vi "configuration UI.vi"() -> ()   [LabVIEW 2015, in "Scan Engine editor node.lvclass"]
uses:
  Scan Engine editor node.lvclass
  <vilib>/NI/Configuration Framework/Node/NodeRef.ctl
  <vilib>/NI/Configuration Framework/Node/NISE_CEF_Node.lvclass
  <vilib>/NI/AMC/Message Queue.ctl
  <vilib>/NI/AMC/Message.ctl
  <vilib>/NI/Tools/Keyed Array/KeyedArray.ctl
  <vilib>/NI/Configuration Framework/Node/UserEventRef.ctl
  <vilib>/NI/Configuration Framework/Controls/EventCluster.ctl
  <vilib>/NI/DCAF UI Toolkit/Controls/Configure.ctl
  <vilib>/NI/DCAF UI Toolkit/Controls/Add.ctl
  <vilib>/NI/DCAF UI Toolkit/Controls/Remove.ctl
  <vilib>/NI/Configuration Framework/Node/StopEvent.ctl
  <vilib>/NI/Configuration Framework/Node/RefreshUIEvent.ctl
  <vilib>/NI/Configuration Framework/Node/CacheState.ctl
  <vilib>/NI/Configuration Framework/Node/NodeChangeEvent.ctl
  <vilib>/NI/Tag Bus/tag/Data Type.ctl
  Permissions Enum.ctl
  <vilib>/NI/DCAF/Tag Editor Core/Table API/Available Tag Menu/channel action event.ctl
  <vilib>/NI/DCAF/Tag Editor Core/Table API/Available Tag Menu/dialog output action.ctl
  <vilib>/NI/Tag Bus Module Framework/channel/TBM channel.lvclass
  <vilib>/NI/Tag Bus/tag/tag descriptor.lvclass
  <vilib>/NI/DCAF/Tag Editor Core/Table API/Table Manager/Call Back Ref Type Def.ctl
  <vilib>/NI/DCAF/Tag Editor Core/Configuration Editor/Classes/Engine Parent/Engine Parent Editor Node.lvclass
  <vilib>/NI/DCAF/Tag Editor Core/Configuration Editor/Classes/Module editor node/module editor node.lvclass
  <vilib>/NI/DCAF UI Toolkit/Controls/Import.ctl
  <vilib>/NI/DCAF UI Toolkit/Controls/Export.ctl
  <vilib>/NI/DCAF/Tag Editor Core/Table API/Table Manager/references.ctl
  <vilib>/Utility/miscctls.llb/LVPositionTypeDef.ctl
  <vilib>/NI/DCAF/Tag Editor Core/Table API/Listbox/Multi Column Listbox.lvclass
  configuration/Scan Engine configuration.lvclass
  <vilib>/NI/Configuration Framework/NISE_CEF_TreeControl.lvlib
  <vilib>/NI/Tools/Keyed Array/Tools_KeyedArray.lvlib
  <vilib>/NI/AMC/AMC.lvlib
  <vilib>/NI/DCAF/Tag Editor Core/Table API/Table Manager.lvlib
  <vilib>/NI/DCAF/Tag Editor Core/Table API/Table Manager/Table Manager.lvclass
  <vilib>/NI/DCAF UI Toolkit/Controls/DCAF UI Elements.lvlib
panel:
  in  "user event out":refnum<user-event>
  in  "Permissions":T1
  in  "data type":T2
  in  "node change":T3
  in  "cache state":T4
  in  "refresh UI":T5
  in  "stop event":T6
  in  "Tab Control":enum32{"Scan Engine Settings", "Import Export"}(tab)
  in  "Overwrite scan engine config":bool
  in  "Remove Button":T7
  in  "Add Button":T8
  in  "Table":i32(listbox)=13
  in  "settings":T9
  in  "Scan Period (uSec)":u32
  in  "Discover Channels?":bool
  in  "Import":T10
  in  "Generate Tags":bool
  in  "Import from csv":T10
  in  "Export":T11
  in  "user event":T12
  in  "main queue":T13
  in  "node ref":T14
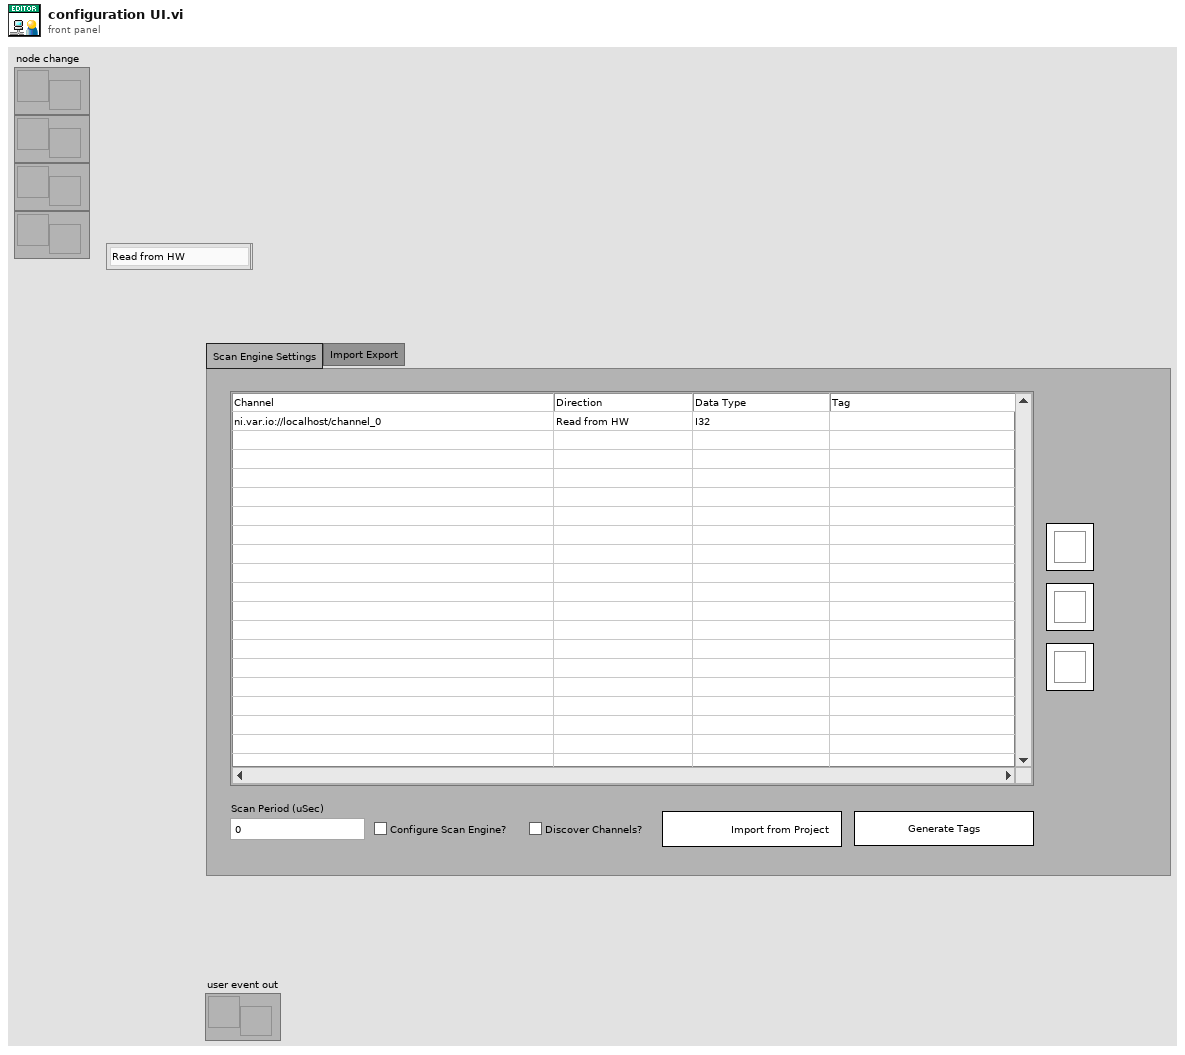
[diagram p1: front panel]
types:
  T1 = typedef "Scan Engine editor node.lvclass/Permissions Enum.ctl" = enum16{"Read from HW", "Write to HW"}
  T2 = typedef "tag bus.lvlib/tag descriptor.lvclass/Data Type.ctl" = enum16{"Double", "Single", "I64", "I32", "I16", "I8", "U64", "U32", "U16", "U8", "Boolean", "String", "Array of Double", "Array of Single", "Array of I64", "Array of I32", "Array of I16", "Array of I8", "Array of U64", "Array of U32", "Array of U16", "Array of U8", "Array of Boolean", "Array of String"}
  T3 = typedef "NISE_CEF_Node.lvclass/NodeChangeEvent.ctl" = refnum<user-event>
  T4 = typedef "NISE_CEF_Node.lvclass/CacheState.ctl" = refnum<user-event>
  T5 = typedef "NISE_CEF_Node.lvclass/RefreshUIEvent.ctl" = refnum<user-event>
  T6 = typedef "NISE_CEF_Node.lvclass/StopEvent.ctl" = refnum<user-event>
  T7 = typedef "DCAF UI Elements.lvlib/Remove.ctl" = bool
  T8 = typedef "DCAF UI Elements.lvlib/Add.ctl" = bool
  T9 = typedef "DCAF UI Elements.lvlib/Configure.ctl" = bool
  T10 = typedef "DCAF UI Elements.lvlib/Import.ctl" = bool
  T11 = typedef "DCAF UI Elements.lvlib/Export.ctl" = bool
  T12 = typedef "NISE_CEF_Node.lvclass/UserEventRef.ctl" = refnum<user-event>
  T13 = typedef "AMC.lvlib/Message Queue.ctl" = refnum<queue>
  T14 = typedef "NISE_CEF_Node.lvclass/NodeRef.ctl" = refnum<data-value>
  T15 = typedef "Table Manager.lvlib/Table Manager.lvclass/references.ctl" = cluster{"stop event":T6, "refresh UI":T5, "cache state":T4, "node change":T3, "user event out":refnum<user-event>, "main queue":T13, "user event":T12}
  T16 = typedef "LVPositionTypeDef.ctl" = cluster{"Left":i32, "Top":i32}
  T17 = typedef "Table Manager.lvlib/Table Manager.lvclass/object ref.ctl" = cluster{"engine":refnum<data-value>, "Node Ref":refnum<data-value>}
  T18 = typedef "Table Manager.lvlib/Column.lvclass/Column Descriptor.ctl" = cluster{"name":string, "caption":string, "Column Type":T19, "Params":string, "AutoSizeMode":i32, "FillWeight":sgl, "MinWidth":u32, "tooltip":string, "Enum Reference":refnum<vi>, "Channel suffix":string, "Read Only":bool, "Call Back VI":T20, "DT Dependency":i32, "name dependency":i32, "data type":T2, "Custom Column":refnum<class "Column.lvclass">}
  T19 = typedef "Table Manager.lvlib/Column.lvclass/Column Type.ctl" = enum16{"String", "Mapping", "Enum", "Custom"}
  T20 = typedef "Table Manager.lvlib/Table Manager.lvclass/Call Back Ref Type Def.ctl" = refnum<vi>
  T21 = typedef "Table Manager.lvlib/Table Manager.lvclass/Table Events.ctl" = cluster{"Menu Selection":refnum<user-event>}
  T22 = enum8{"Enabled", "Disabled", "Disabled and Grayed Out"}
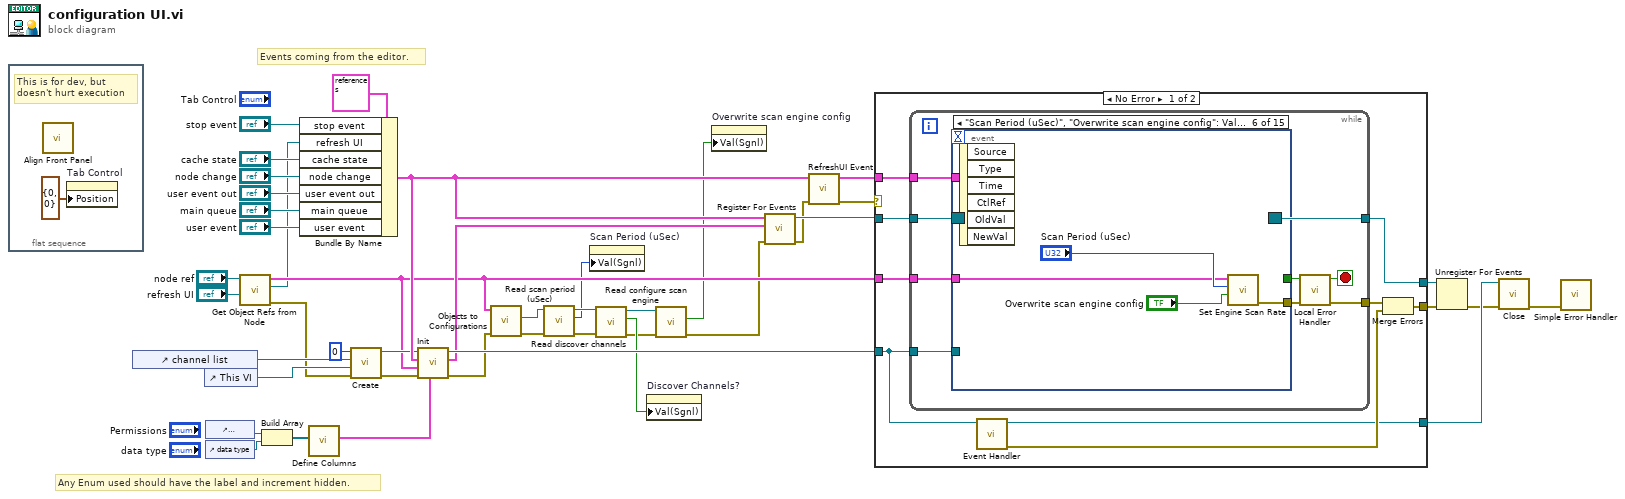
[diagram p0: block diagram]
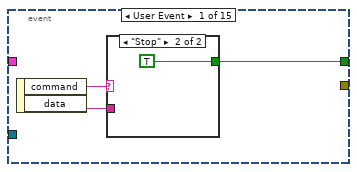
[diagram p2: hidden frame]
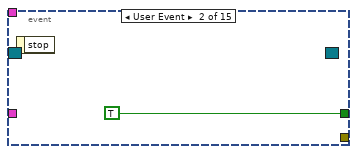
[diagram p4: hidden frame]
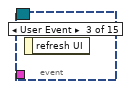
[diagram p5: hidden frame]
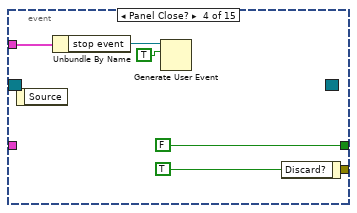
[diagram p6: hidden frame]
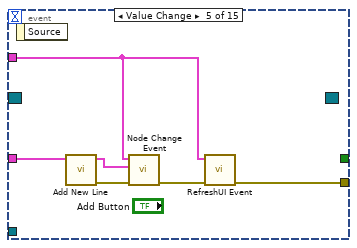
[diagram p7: hidden frame]
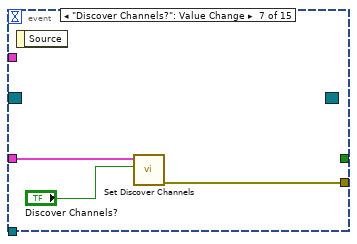
[diagram p8: hidden frame]
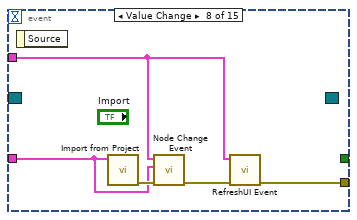
[diagram p9: hidden frame]
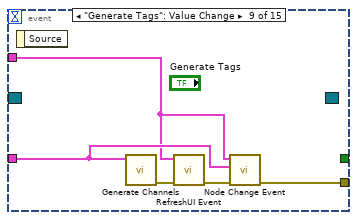
[diagram p10: hidden frame]
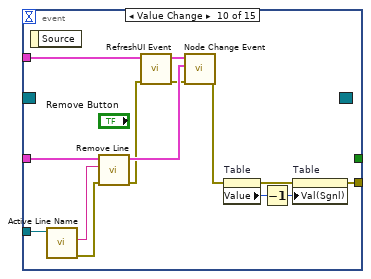
[diagram p11: hidden frame]
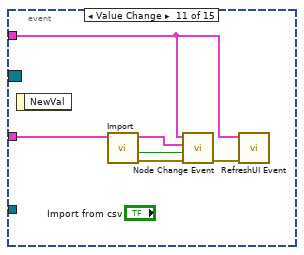
[diagram p12: hidden frame]
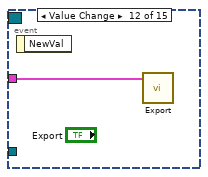
[diagram p13: hidden frame]
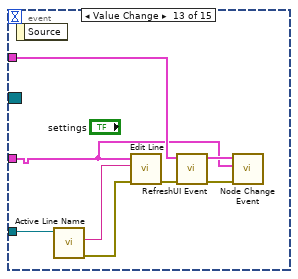
[diagram p14: hidden frame]
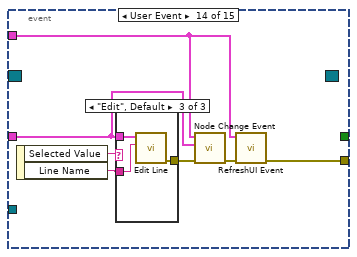
[diagram p15: hidden frame]
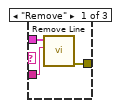
[diagram p16: hidden frame]
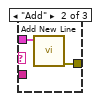
[diagram p17: hidden frame]
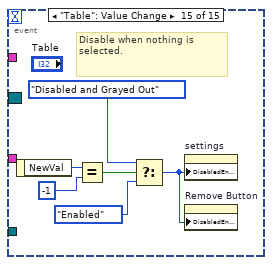
[diagram p18: hidden frame]
diagram:
  # "Any Enum used should have the label and increment hidden."
  # "Events coming from the editor."
  n1 = flat-sequence {
    frame #0 {
      # "This is for dev, but doesn't hurt execution"
      n2 = call <vilib>:"Align Front Panel.vi"() -> ()  [unwired: 10 in, 2 out]
      n3 = property on="Tab Control" class="TabCtl (strict)"("Position"=T16 {"Left"=0, "Top"=0}) -> ()  [unwired: 2 in, 2 out]
    }
  }
  n4 = control-ref of="channel list"() -> (w24:refnum<vi>)
  n5 = control-ref of="This VI"() -> (w22:refnum<vi>)
  n6 = control-ref of="Permissions"() -> (w31:refnum<vi>)
  n7 = control-ref of="data type"() -> (w30:refnum<vi>)
  n8 = call "Get Object Refs from Node.vi"("refresh UI"="refresh UI", "Data Value Reference in"="node ref") -> ("error out"=w6:errorcluster, "refresh UI out"=w7:T5, "references"=w18:T17)  [unwired: 7 in]
  n9 = Build Array(w31, w30) -> (w29:refnum<vi>[])
  n10 = Bundle By Name(cluster=T15 {"stop event"=refnum, "refresh UI"=refnum, "cache state"=refnum, "node change"=refnum, "user event out"=refnum, "main queue"=refnum, "user event"=refnum} ("References"), "stop event"="stop event", "refresh UI"=w7, "cache state"="cache state", "node change"="node change", "user event out"="user event out", "main queue"="main queue", "user event"="user event") -> (w32:T15)
  n11 = call "Define Columns.vi"("Enum Array"=w29) -> ("Column Definition"=w34:T18[])  [unwired: 10 in]
  n12 = call <vilib>:"Create.vi"("error in (no error)"=w6, "Top VI"=w22, "Listbox"=w24, "Index"=0) -> ("error out"=w5:errorcluster, "reference out"=w21:refnum<class "Multi Column Listbox.lvclass">)  [unwired: 6 in]
  n13 = call-dynamic "Init.vi"("Column Descriptors"=w34, "error in (no error)"=w5, "Node object refs"=w18, "Event References"=w32, "Multi Column Listbox in"=w21) -> ("error out"=w20:errorcluster, "Table Events"=w19:T21, "Multi Column Listbox out"=w28:refnum<class "Multi Column Listbox.lvclass">)  [unwired: 4 in]
  n14 = call "Objects to Configurations.vi"("error in (no error)"=w20, "Objects in"=w18) -> ("error out"=w14:errorcluster, "tag bus configurable plugin module configuration"=w17:refnum<class "Scan Engine configuration.lvclass">)  [unwired: 7 in, 1 out]
  n15 = call-dynamic "Read scan period (uSec).vi"("error in (no error)"=w14, "Scan Engine configuration1 in"=w17) -> ("error out"=w15:errorcluster, "scan period (uSec)"=w13:u32, "Scan Engine configuration1 out"=w16:refnum<class "Scan Engine configuration.lvclass">)  [unwired: 7 in]
  n16 = property on="Scan Period (uSec)" class="DigNum (strict)"("Val(Sgnl)"=w13) -> ()  [unwired: 2 in, 2 out]
  n17 = call-dynamic "Read discover channels.vi"("error in (no error)"=w15, "Scan Engine configuration1 in"=w16) -> ("error out"=w4:errorcluster, "discover channels"=w12:bool, "Scan Engine configuration1 out"=w3:refnum<class "Scan Engine configuration.lvclass">)  [unwired: 7 in]
  n18 = property on="Discover Channels?" class="Bool (strict)"("Val(Sgnl)"=w12) -> ()  [unwired: 2 in, 2 out]
  n19 = call-dynamic "Read configure scan engine.vi"("error in (no error)"=w4, "Scan Engine configuration1 in"=w3) -> ("error out"=w2:errorcluster, "configure scan engine"=w1:bool)  [unwired: 7 in, 1 out]
  n20 = property on="Overwrite scan engine config" class="Bool (strict)"("Val(Sgnl)"=w1) -> ()  [unwired: 2 in, 2 out]
  n21 = call "Register For Events.vi"("error in"=w2, "Table Events"=w19, "References"=w32) -> ("error out"=w26:errorcluster, "Event Registration Refnum"=w35:refnum<event-registration>)  [unwired: 7 in]
  n22 = call "RefreshUI Event.vi"("error in (no error)"=w26, "References in"=w32) -> ("error out"=w25:errorcluster, "References out"=w33:T15)  [unwired: 8 in]
  n23 = case shown="No Error" w25 {
    selector: w25 -> [_ w147]
    tunnel: w35 -> [w54 w146]
    tunnel: [w53 w146] -> w44
    tunnel: [w47 w147] -> w43
    tunnel: w33 -> [w52 _]
    tunnel: w18 -> [w51 _]
    tunnel: w28 -> [w50 w145]
    tunnel: [w46 w145] -> w11
    frame No Error {
      n24 = while {
        tunnel: w54 -> [w63]
        tunnel: [w62] -> w53
        tunnel: [w59] -> w48
        tunnel: w52 -> [w57]
        tunnel: w51 -> [w56]
        tunnel: w50 -> [w55]
        stop <- w61 stop-if-true
        n25 = event shown="[5] \"Scan Period (uSec)\", \"Overwrite scan engine config\": Value Change" {
          selector: w63 -> [_ _ _ _ _ _ _ _ _ _ _ _ _ _ _]
          dyn-events: [_ _ _ _ _ _ _ _ _ _ _ _ _ _ _] -> w62
          timeout: _ -> [_ _ _ _ _ _ _ _ _ _ _ _ _ _ _]
          tunnel: [w66 TRUE _ FALSE _ _ _ _ _ _ _ _ _ _ _] -> w60
          tunnel: [_ _ _ _ w74 w80 w83 w88 w91 w96 _ _ _ w128 _] -> w58
          tunnel: w57 -> [_ _ _ w70 w77 _ _ w87 w92 w108 w110 _ w118 w124 _]
          tunnel: w56 -> [_ _ _ _ w78 w81 w85 w86 w93 w107 w114 w115 w117 w125 _]
          tunnel: w55 -> [_ _ _ _ _ _ _ _ _ w103 _ _ w123 _ _]
          event User Event {
            n26 = event-data() -> ("command"=w65:string, "data"=w64:string)  [unwired: 1 in]
            n27 = case shown="\"Stop\"" w65 {
              tunnel: [_ TRUE] -> w66
              tunnel: w64 -> [_ _]
              frame Default {
              }
              frame "Stop" {
              }
            }
          }
          event User Event {
            n28 = event-data() -> ()  [unwired: 1 in, 1 out]
          }
          event User Event {
            n29 = event-data() -> ()  [unwired: 1 in, 1 out]
          }
          event Panel Close? {
            n30 = event-data() -> ()  [unwired: 1 in, 1 out]
            n31 = Unbundle By Name(w70) -> ("stop event"=w69:T6)
            n32 = Generate User Event(user event=w69, event data cluster=TRUE ("event data")) -> ()  [unwired: 2 in, 2 out]
            n33 = event-data("Discard?"=TRUE) -> ()  [unwired: 1 in, 1 out]
          }
          event Value Change {
            n34 = event-data() -> ()  [unwired: 1 in, 1 out]
            n35 = call "Add New Line.vi"("objects"=w78) -> ("error out"=w76:errorcluster)  [unwired: 9 in, 1 out]
            n36 = call "Node Change Event.vi"("error in (no error)"=w76, "objects"=w78, "References in"=w77) -> ("error out"=w75:errorcluster)  [unwired: 8 in]
            n37 = call "RefreshUI Event.vi"("error in (no error)"=w75, "References in"=w77) -> ("error out"=w74:errorcluster)  [unwired: 8 in, 1 out]
          }
          event "Scan Period (uSec)", "Overwrite scan engine config": Value Change {
            n38 = event-data() -> ()  [unwired: 1 in, 6 out]
            n39 = call "Set Engine Scan Rate.vi"("Configure Scan Engine"="Overwrite scan engine config", "scan period (uSec)"="Scan Period (uSec)", "references in"=w81) -> ("error out"=w80:errorcluster)  [unwired: 7 in, 1 out]
          }
          event "Discover Channels?": Value Change {
            n40 = event-data() -> ()  [unwired: 1 in, 1 out]
            n41 = call "Set Discover Channels.vi"("discover channels"="Discover Channels?", "references in"=w85) -> ("error out"=w83:errorcluster)  [unwired: 8 in, 1 out]
          }
          event Value Change {
            n42 = event-data() -> ()  [unwired: 1 in, 1 out]
            n43 = call "Import from Project.vi"("references"=w86) -> ("error out"=w90:errorcluster)  [unwired: 9 in, 1 out]
            n44 = call "Node Change Event.vi"("error in (no error)"=w90, "objects"=w86, "References in"=w87) -> ("error out"=w89:errorcluster)  [unwired: 8 in]
            n45 = call "RefreshUI Event.vi"("error in (no error)"=w89, "References in"=w87) -> ("error out"=w88:errorcluster)  [unwired: 8 in, 1 out]
          }
          event "Generate Tags": Value Change {
            n46 = event-data() -> ()  [unwired: 1 in, 1 out]
            n47 = call "Generate Channels.vi"("references in"=w93) -> ("error out"=w94:errorcluster)  [unwired: 10 in]
            n48 = call "RefreshUI Event.vi"("error in (no error)"=w94, "References in"=w92) -> ("error out"=w95:errorcluster)  [unwired: 8 in, 1 out]
            n49 = call "Node Change Event.vi"("error in (no error)"=w95, "objects"=w93, "References in"=w92) -> ("error out"=w91:errorcluster)  [unwired: 8 in]
          }
          event Value Change {
            n50 = event-data() -> ()  [unwired: 1 in, 1 out]
            n51 = call-dynamic "Active Line Name.vi"("Multi Column Listbox in"=w103) -> ("error out"=w101:errorcluster, "Active Line Name"=w102:string)  [unwired: 8 in, 1 out]
            n52 = call "Remove Line.vi"("error in"=w101, "Active Line Name"=w102, "Objects"=w107) -> ("error out"=w104:errorcluster)  [unwired: 8 in]
            n53 = call "RefreshUI Event.vi"("error in (no error)"=w104, "References in"=w108) -> ("error out"=w106:errorcluster, "References out"=w105:T15)  [unwired: 8 in]
            n54 = call "Node Change Event.vi"("error in (no error)"=w106, "objects"=w107, "References in"=w105) -> ("error out"=w98:errorcluster)  [unwired: 8 in]
            n55 = property on="Table" class="MCListbox (strict)"(error in=w98) -> (error out=w97:errorcluster, "Value"=w100:i32)  [unwired: 1 in, 1 out]
            n56 = Decrement(x=w100) -> (x-1=w99:i32)
            n57 = property on="Table" class="MCListbox (strict)"(error in=w97, "Val(Sgnl)"=w99) -> (error out=w96:errorcluster)  [unwired: 1 in, 1 out]
          }
          event Value Change {
            n58 = event-data() -> ()  [unwired: 1 in, 1 out]
            n59 = call "Import.vi"("Objects in"=w114) -> ("error out"=w113:errorcluster, "Update"=w112:bool, "Objects out"=w111:T17)  [unwired: 8 in]
            n60 = call "Node Change Event.vi"("error in (no error)"=w113, "Send (T)"=w112, "objects"=w111, "References in"=w110) -> ("error out"=w109:errorcluster)  [unwired: 7 in]
            n61 = call "RefreshUI Event.vi"("error in (no error)"=w109, "References in"=w110) -> ()  [unwired: 8 in, 2 out]
          }
          event Value Change {
            n62 = event-data() -> ()  [unwired: 1 in, 1 out]
            n63 = call "Export.vi"("Objects"=w115) -> ()  [unwired: 10 in, 1 out]
          }
          event Value Change {
            n64 = event-data() -> ()  [unwired: 1 in, 1 out]
            n65 = call-dynamic "Active Line Name.vi"("Multi Column Listbox in"=w123) -> ("error out"=w121:errorcluster, "Active Line Name"=w122:string)  [unwired: 8 in, 1 out]
            n66 = call "Edit Line.vi"("error in"=w121, "Line Name"=w122, "References"=w117) -> ("error out"=w116:errorcluster)  [unwired: 7 in, 1 out]
            n67 = call "RefreshUI Event.vi"("error in (no error)"=w116, "References in"=w118) -> ("error out"=w119:errorcluster, "References out"=w120:T15)  [unwired: 8 in]
            n68 = call "Node Change Event.vi"("error in (no error)"=w119, "objects"=w117, "References in"=w120) -> ()  [unwired: 8 in, 1 out]
          }
          event User Event {
            n69 = event-data() -> ("Selected Value"=w130:string, "Line Name"=w127:string)  [unwired: 1 in]
            n70 = case shown="\"Edit\", Default" w130 {
              tunnel: w127 -> [w133 _ w138]
              tunnel: w125 -> [w132 w135 w137]
              tunnel: [w131 w134 w136] -> w126
              frame "Remove" {
                n71 = call "Remove Line.vi"("Active Line Name"=w133, "Objects"=w132) -> ("error out"=w131:errorcluster)  [unwired: 9 in]
              }
              frame "Add" {
                n72 = call "Add New Line.vi"("objects"=w135) -> ("error out"=w134:errorcluster)  [unwired: 9 in, 1 out]
              }
              frame "Edit", Default {
                n73 = call "Edit Line.vi"("Line Name"=w138, "References"=w137) -> ("error out"=w136:errorcluster)  [unwired: 8 in, 1 out]
              }
            }
            n74 = call "Node Change Event.vi"("error in (no error)"=w126, "objects"=w125, "References in"=w124) -> ("error out"=w129:errorcluster)  [unwired: 8 in]
            n75 = call "RefreshUI Event.vi"("error in (no error)"=w129, "References in"=w124) -> ("error out"=w128:errorcluster)  [unwired: 8 in, 1 out]
          }
          event "Table": Value Change {
            # "Disable when nothing is selected."
            n76 = event-data() -> ("NewVal"=w144:i32)  [unwired: 1 in]
            n77 = Equal?(x=w144, y=-1) -> (x = y?=w142:bool)
            n78 = Select(t=T22."Disabled and Grayed Out" ("Disabled"), s=w142, f=T22."Enabled" ("Disabled")) -> (s? t:f=w140:T22)
            n79 = property on="settings" class="Bool"("DisabledEnum"=w140) -> ()  [unwired: 2 in, 2 out]
            n80 = property on="Remove Button" class="Bool"("DisabledEnum"=w140) -> ()  [unwired: 2 in, 2 out]
          }
        }
        n81 = call "Local Error Handler.vi"("error in"=w58, "Stop in"=w60) -> ("error out"=w59:errorcluster, "Stop out"=w61:bool)  [unwired: 8 in]
      }
      n82 = call-dynamic "Event Handler.vi"("Listbox in"=w50) -> ("error out"=w49:errorcluster, "Listbox out"=w46:refnum<class "Multi Column Listbox.lvclass">)  [unwired: 9 in]
      n83 = Merge Errors(w48, w49) -> (w47:errorcluster)
    }
    frame Error {
    }
  }
  n84 = Unregister For Events(event registration refnum=w44, error in=w43) -> (error out=w10:errorcluster)
  n85 = call-dynamic "Close.vi"("error in (no error)"=w10, "Multi Column Listbox in"=w11) -> ("error out"=w9:errorcluster)  [unwired: 8 in, 1 out]
  n86 = call <vilib>:"Simple Error Handler.vi"("error in (no error)"=w9) -> ()  [unwired: 4 in, 5 out]
